vi "SetStringInfo.vi"(0 "reference":refnum<class "ChoiceNode.lvclass">, 1 "State":string, 2 "Action":string, 5 "error in (no error)":errorcluster) -> (14 "reference out":refnum<class "ChoiceNode.lvclass">, 19 "error out":errorcluster)   [LabVIEW 2020, in "ChoiceNode.lvclass"]
uses:
  <resource>/Framework/Providers/Open_GDS/UML/ChoiceNode_class/ChoiceNode.lvclass
  <resource>/Framework/Providers/Open_GDS/UML/MultiLineString_class/MultiLineString.lvclass
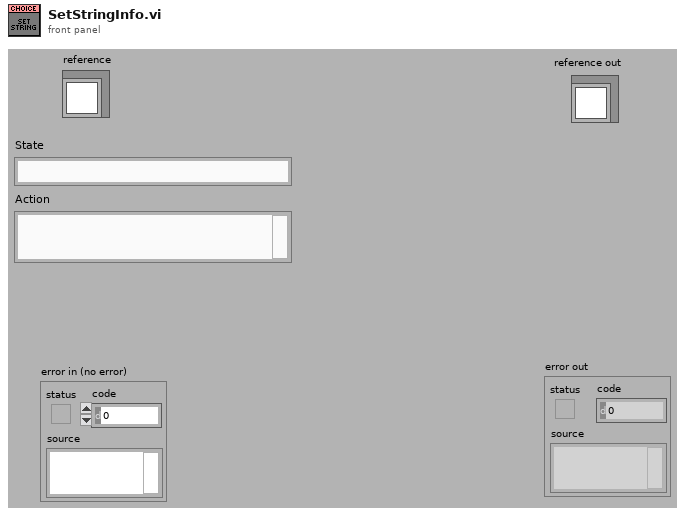
[diagram p1: front panel]
types:
  T1 = typedef "ChoiceNode.lvclass/ObjectAttributes.ctl" = cluster{"Text":refnum<class "MultiLineString.lvclass">, "DEFAULT_WIDTH":i32, "DEFAULT_HEIGHT":i32}
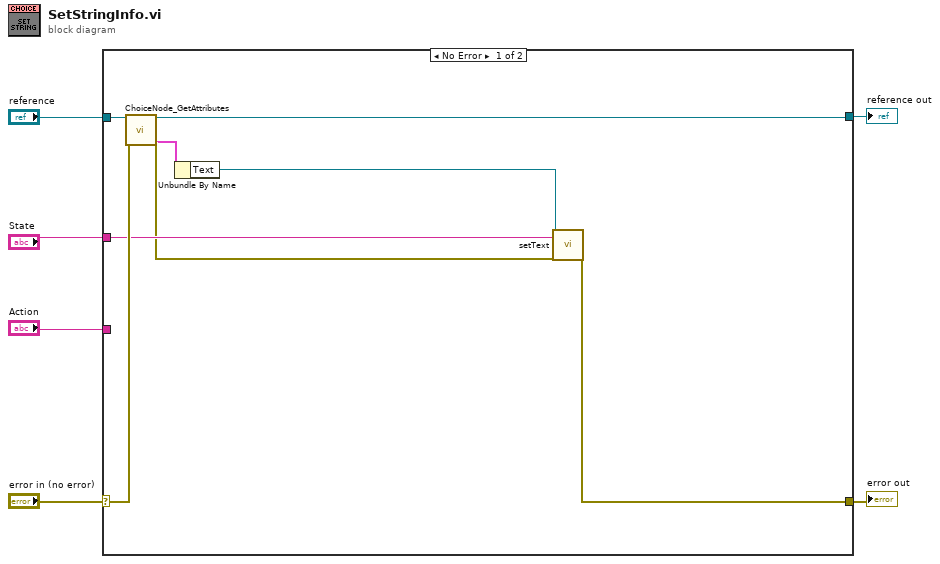
[diagram p0: block diagram]
diagram:
  n1 = case shown="No Error" "error in (no error)" {
    selector: "error in (no error)" -> [w14 w15]
    tunnel: "reference" -> [w13 w16]
    tunnel: [w10 w15] -> w4
    tunnel: [w12 w16] -> w3
    tunnel: "State" -> [w9 _]
    tunnel: "Action" -> [_ _]
    frame No Error {
      n2 = call <resource>:"ChoiceNode_GetAttributes.vi"("reference in"=w13, "error in (no error)"=w14) -> ("reference out"=w12:refnum<class "ChoiceNode.lvclass">, "Data"=w7:T1, "error out"=w8:errorcluster)  [unwired: 1 in, 14 out]
      n3 = Unbundle By Name(w7) -> ("Text"=w11:refnum<class "MultiLineString.lvclass">)
      n4 = call-dynamic "setText.vi"("reference"=w11, "text"=w9, "error in (no error)"=w8) -> ("error out"=w10:errorcluster)  [unwired: 16 out]
    }
    frame Error {
    }
  }
  "reference out" <- w3
  "error out" <- w4
